vi "Run Unit Tests.vi"   [LabVIEW 2020]
doc: "Runs the Caraya unit tests in this folder (every *.utest.vi) from the command line through G-CLI, and writes a JUnit XML report.\n\nUsage: g-cli --lv-ver 2020 \"<path>\\Run Unit Tests.vi\" -- [report path]\n\nThe report path defaults to Unit Tests-TestReport.xml in this folder. The exit code is 0 when every test passes and the Caraya error code (7002) when a test fails."
uses:
  <vilib>/addons/_JKI Toolkits/Caraya/classes/Test Report.JUnit/Test Report.JUnit.lvclass
  C:/Program Files (x86)/National Instruments/LabVIEW 2020/vi.lib/addons/_JKI Toolkits/Caraya/classes/Test Report/Test Report.lvclass
  <vilib>/Wiresmith Technology/G CLI/CLI Class/CLI.lvclass
  <vilib>/addons/_JKI Toolkits/Caraya/Caraya.lvlib
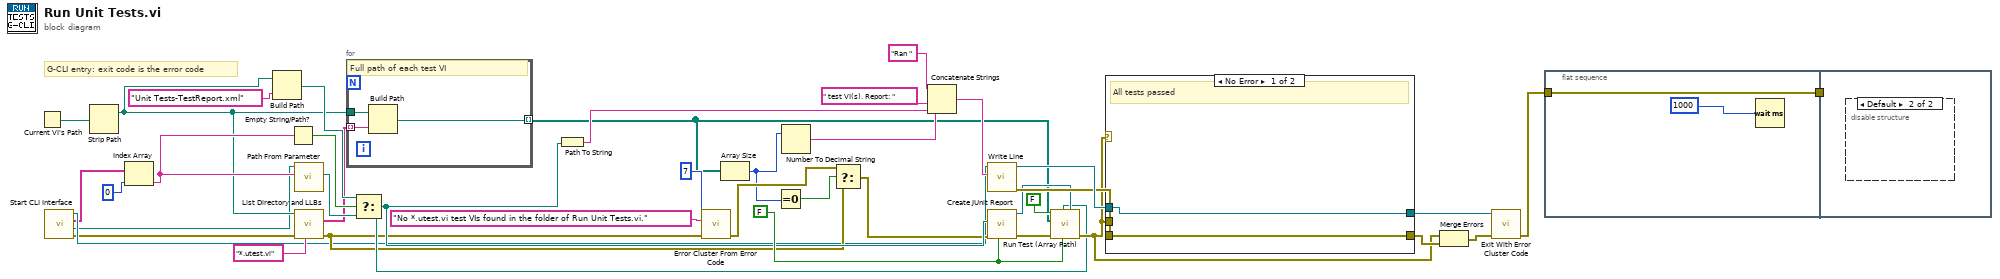
[diagram p0: block diagram]
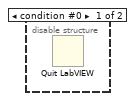
[diagram p2: hidden frame]
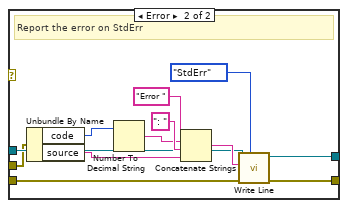
[diagram p3: hidden frame]
diagram:
  w24 = FALSE ("Verbose")
  # "G-CLI entry: exit code is the error code"
  n1 = Current VI's Path() -> (path=w5:path)
  n2 = call <vilib>:"Start CLI Interface.vi"() -> ("error out"=w1:errorcluster, "Working Directory"=w2:path, "Custom Parameters"=w3:string[], "CLI out"=w4:refnum<class "CLI.lvclass">)  [unwired: 8 in]
  n3 = Strip Path(path=w5) -> (stripped path=w6:path)  [unwired: 1 out]
  n4 = Index Array(array=w3, index=0) -> (element=w18:string)
  n5 = Build Path(base path=w6, name or relative path="Unit Tests-TestReport.xml" ("default report name")) -> (appended path=w22:path)
  n6 = Empty String/Path?(string/path=w18) -> (empty?=w19:bool)
  n7 = call <vilib>:"Path From Parameter.vi"("Path Parameter"=w18, "Working Directory"=w2) -> ("Full Path"=w20:path)  [unwired: 9 in]
  n8 = call <vilib>:"List Directory and LLBs.vi"("pattern"="*.utest.vi", "error in (no error)"=w1, "Folder Path"=w6) -> ("error out"=w9:errorcluster, "Files sans LLBs"=w8:string[])  [unwired: 5 in, 2 out]
  n9 = for {
    tunnel: w6 -> [w42]
    tunnel: w8 -> [w41] mode=indexing
    tunnel: [w43] -> w10 mode=indexing
    # "Full path of each test VI"
    n10 = Build Path(base path=w42, name or relative path=w41) -> (appended path=w43:path)
  }
  n11 = Select(t=w22, s=w19, f=w20) -> (s? t:f=w23:path)
  n12 = Path To String(path=w23) -> (string=w32:string)
  n13 = call <vilib>:"Error Cluster From Error Code.vi"("error in (no error)"=w9, "error message (\"\")"="No *.utest.vi test VIs found in the folder of Run Unit Tests.vi." ("error message"), "error code (0)"=7) -> ("error out"=w15:errorcluster)  [unwired: 6 in]
  n14 = Array Size(array=w10) -> (size(s)=w11:i32)
  n15 = Equal To 0?(x=w11) -> (x = 0?=w12:bool)
  n16 = Number To Decimal String(number=w11) -> (decimal integer string=w30:string)  [unwired: 1 in]
  n17 = Select(t=w15, s=w12, f=w9) -> (s? t:f=w16:errorcluster)
  n18 = Concatenate Strings("Ran " ("prefix"), w30, " test VI(s). Report: " ("middle"), w32) -> (w33:string)
  n19 = call <vilib>:"Write Line.vi"("Text to Write"=w33, "CLI in"=w4) -> ("error out"=w34:errorcluster, "CLI out"=w35:refnum<class "CLI.lvclass">)  [unwired: 8 in]
  n20 = call <vilib>:"Create JUnit Report.vi"("Verbose"=w24, "error in (no error)"=w16, "Report Path"=w23) -> ("error out"=w25:errorcluster, "Test Report.JUnit out"=w26:refnum<class "Test Report.JUnit.lvclass">)  [unwired: 7 in]
  n21 = call <vilib>:"Run Test (Array Path).vi"("Test Report"=w26, "Verbose"=w24, "Report Path"=w23, "error in"=w25, "Paths"=w10, "Interactive (T)"=FALSE) -> ("error out"=w28:errorcluster)  [unwired: 4 in, 1 out]
  n22 = case shown="No Error" w28 {
    tunnel: w35 -> [w44 w47]
    tunnel: w34 -> [w45 w48]
    tunnel: w28 -> [_ w46]
    tunnel: [w44 w57] -> w36
    tunnel: [w45 w56] -> w37
    frame No Error {
      # "All tests passed"
    }
    frame Error {
      # "Report the error on StdErr"
      n23 = Unbundle By Name(w46) -> ("code"=w49:i32, "source"=w50:string)
      n24 = Number To Decimal String(number=w49) -> (decimal integer string=w52:string)  [unwired: 1 in]
      n25 = Concatenate Strings("Error " ("error prefix"), w52, ": " ("separator"), w50) -> (w54:string)
      n26 = call <vilib>:"Write Line.vi"("Output (StdOut)"=enum16{"StdOut", "StdErr"}."StdErr", "error in (no error)"=w48, "Text to Write"=w54, "CLI in"=w47) -> ("error out"=w56:errorcluster, "CLI out"=w57:refnum<class "CLI.lvclass">)  [unwired: 6 in]
    }
  }
  n27 = Merge Errors(w28, w37) -> (w38:errorcluster)
  n28 = call <vilib>:"Exit With Error Cluster Code.vi"("error in (no error)"=w38, "CLI in"=w36) -> ("error out"=w39:errorcluster)  [unwired: 9 in]
  n29 = flat-sequence {
    tunnel: w39 -> [w59]
    tunnel: [w59] -> w40
    tunnel: w40 -> [_]
    frame #0 {
      n30 = Wait (ms)(milliseconds to wait=u32 1000) -> ()  [unwired: 1 out]
    }
    frame #1 {
      n31 = disable-structure shown="Default" {
        frame condition #0 {
          n32 = Quit LabVIEW() -> ()  [unwired: 1 in]
        }
        frame condition #1 (active) {
        }
      }
    }
  }
